vi "CompVisionUtil_EstimateCameraToTarget.vi"(9 "GyroAngle":T1={"VALUE"=0.0, "COS"=1.0, "SIN"=0.0} {"SIN" format="%13.4f"; "COS" format="%13.4f"; "VALUE" format="%13.4f"}, 10 "FieldToTarget":T6={"Translation3d"={"X"=0.0, "Y"=0.0, "Z"=0.0}, "Rotation3d"={"Q_quaternion"={"R"=1.0, "V"=[0.0, 0.0, 0.0]}}} {"Translation3d"."Z" format="%14.3f"; "Translation3d"."Y" format="%14.3f"; "Translation3d"."X" format="%14.3f"}, 11 "CameraToTargetTranslation":T3 {"Z" format="%14.3f"; "Y" format="%14.3f"; "X" format="%14.3f"}) -> (3 "EstimateCameraToTarget":T2={"TRANSLATION3D"={"X"=0.0, "Y"=0.0, "Z"=0.0}, "ROTATION3D"={"Q_quaternion"={"R"=1.0, "V"=[0.0, 0.0, 0.0]}}, "XF"=FALSE} {"TRANSLATION3D"."Z" format="%14.3f"; "TRANSLATION3D"."Y" format="%14.3f"; "TRANSLATION3D"."X" format="%14.3f"})   [LabVIEW 2019, in "Trajectory_Library.lvlib"]
doc: "Estimates a Transform2d that maps the camera position to the target position, using the robot's gyro. Note that the gyro angle provided *must* line up with the field coordinate system -- that is, it should read zero degrees when pointed towards the opposing alliance station, and increase as the robot rotates CCW.\n \nInputs: \n - CameraToTargetTranslation -- A Translation3d that encodes the x/y position \n of the target relative to the camera.\n - FieldToTarget -- A Pose3d representing the target position in the field coordinate \n system.\n - GyroAngle -- A rotation2d representing the current robot gyro angle, likely from odometry.\n\nOutputs:\n - EstimateCameraToTarget -- A Transform3d that takes us from the camera to \n the target."
uses:
  Trajectory_Library.lvlib
  TypeDef/ROTATION2D.ctl
  TypeDef/TRANSLATION3D.ctl
  TypeDef/QUATERNION.ctl
  TypeDef/ROTATION3D.ctl
  TypeDef/TRANSFORM3D.ctl
  TypeDef/POSE3D.ctl
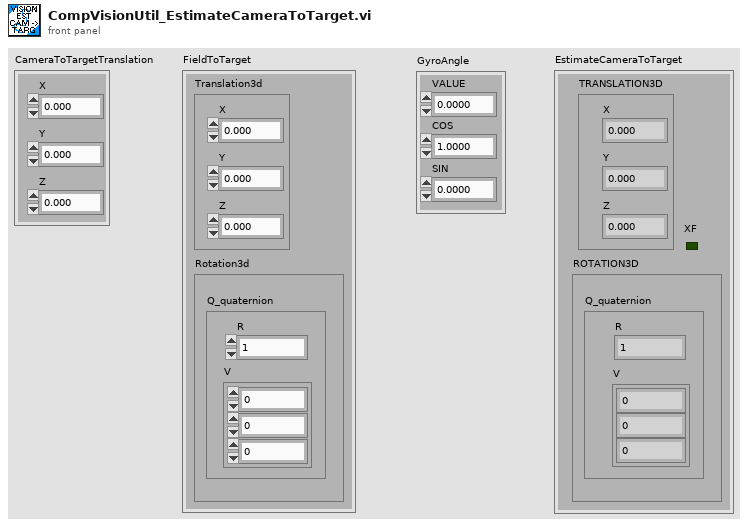
[diagram p1: front panel]
types:
  T1 = typedef "Trajectory_Library.lvlib/ROTATION2D.ctl" = cluster{"VALUE":dbl, "COS":dbl, "SIN":dbl}
  T2 = typedef "Trajectory_Library.lvlib/TRANSFORM3D.ctl" = cluster{"TRANSLATION3D":T3, "ROTATION3D":T4, "XF":bool}
  T3 = typedef "Trajectory_Library.lvlib/TRANSLATION3D.ctl" = cluster{"X":dbl, "Y":dbl, "Z":dbl}
  T4 = typedef "Trajectory_Library.lvlib/ROTATION3D.ctl" = cluster{"Q_quaternion":T5}
  T5 = typedef "Trajectory_Library.lvlib/QUATERNION.ctl" = cluster{"R":dbl, "V":dbl[]}
  T6 = typedef "Trajectory_Library.lvlib/POSE3D.ctl" = cluster{"Translation3d":T3, "Rotation3d":T4}
  T7 = typedef "WPILib_Math.lvlib/ROTATION3D.ctl" = cluster{"Q_quaternion":T8}
  T8 = typedef "WPILib_Math.lvlib/QUATERNION.ctl" = cluster{"R":dbl, "V":dbl[]}
  T9 = typedef "WPILib_Math.lvlib/TRANSFORM3D.ctl" = cluster{"TRANSLATION3D":T10, "ROTATION3D":T7, "XF":bool}
  T10 = typedef "WPILib_Math.lvlib/TRANSLATION3D.ctl" = cluster{"X":dbl, "Y":dbl, "Z":dbl}
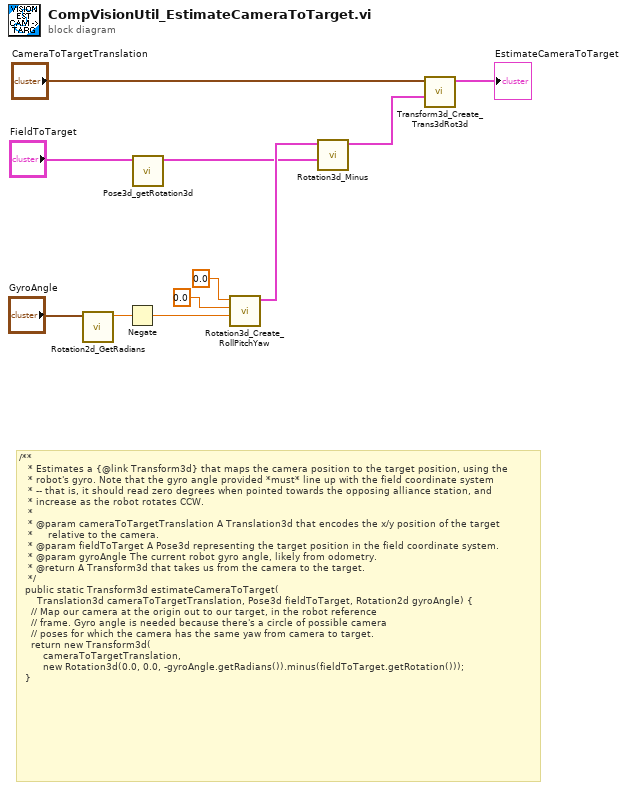
[diagram p0: block diagram]
diagram:
  # "/**\n   * Estimates a {@link Transform3d} that maps the camera position to the target position, using the\n   * robot's gyro. Note that the gyro angle provided *must* line up with the field coordinate system\n   * -- that is, it should read zero degrees when pointed towards the opposing alliance station, and\n   * increase as the robot rotates CCW.\n   *\n   * @param cameraToTargetTranslation A Translation3d that encodes the x/y position of the target\n   *     relative to the camera.\n   * @param fieldToTarget A Pose3d representing the target position in the field coordinate system.\n   * @param gyroAngle The current robot gyro angle, likely from odometry.\n   * @return A Transform3d that takes us from the camera to the target.\n   */\n  public static Transform3d estimateCameraToTarget(\n      Translation3d cameraToTargetTranslation, Pose3d fieldToTarget, Rotation2d gyroAngle) {\n    // Map our camera at the origin out to our target, in the robot reference\n    // frame. Gyro angle is needed because there's a circle of possible camera\n    // poses for which the camera has the same yaw from camera to target.\n    return new Transform3d(\n        cameraToTargetTranslation,\n        new Rotation3d(0.0, 0.0, -gyroAngle.getRadians()).minus(fieldToTarget.getRotation()));\n  }"
  n1 = call "Rotation2d_GetRadians.vi"("in ROTATION"="GyroAngle") -> ("AngleRadians"=w9:dbl)  [unwired: 10 in]
  n2 = Negate(x=w9) -> (-x=w8:dbl)
  n3 = call "Pose3d_getRotation3d.vi"("in Pose3d"="FieldToTarget") -> ("out Rotation3d"=w2:T7)  [unwired: 10 in]
  n4 = call "Rotation3d_Create_RollPitchYaw.vi"("Yaw"=w8, "Pitch"=0.0, "Roll"=0.0) -> ("Rotation3d"=w3:T4)  [unwired: 8 in]
  n5 = call "Rotation3d_Minus.vi"("other Rotation3d"=w2, "in Rotation3d"=w3) -> ("out Rotation3d"=w1:T4)  [unwired: 9 in]
  n6 = call "Transform3d_Create_Trans3dRot3d.vi"("Rotation3d"=w1, "Translation3d"="CameraToTargetTranslation") -> ("Transform3d"=→"EstimateCameraToTarget":T9)  [unwired: 9 in]
